vi "FRC_read utility images.vi"(7 "utilities data array":T1[](array[typedef])) -> (8 "menu array":cluster{"button":bool, "picture":picture}[](array[cluster]), 10 "names":string[](array[string]))   [LabVIEW 2023, in "GettingStartedWindow.lvlib"]
uses:
  <resource>/modes/FRC/GettingStartedWindow.lvlib
  <resource>/modes/FRC/FRC_UtilitiesData.ctl
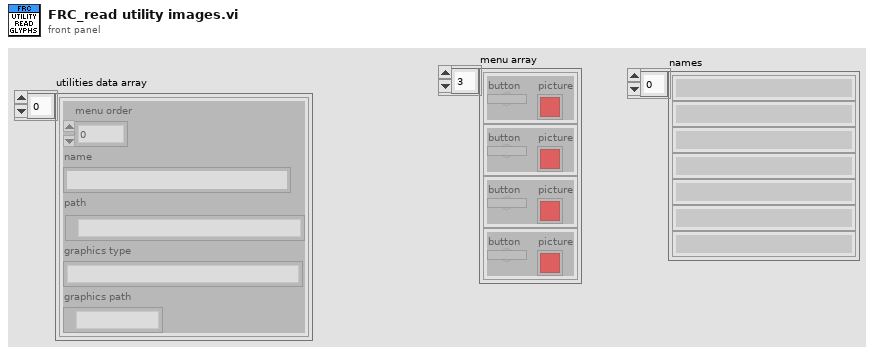
[diagram p1: front panel]
types:
  T1 = typedef "GettingStartedWindow.lvlib/FRC_UtilitiesData.ctl" = cluster{"menu order":i32, "name":string, "path":path, "graphics type":string, "graphics path":path}
  T2 = typedef "imagedata.ctl" = cluster{"image type":i32, "image depth":i32, "image":u8[], "mask":u8[], "colors":u32[], "Rectangle":cluster{"left":i16, "top":i16, "right":i16, "bottom":i16}}
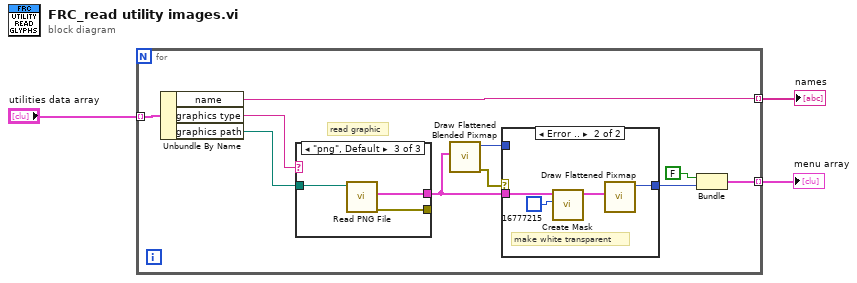
[diagram p0: block diagram]
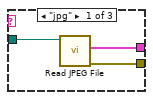
[diagram p3: hidden frame]
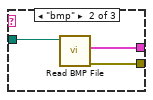
[diagram p4: hidden frame]
diagram:
  n1 = for {
    tunnel: "utilities data array" -> [w13] mode=indexing
    tunnel: [w9] -> w3 mode=indexing
    tunnel: [w8] -> w2 mode=indexing
    # "read graphic"
    n2 = Unbundle By Name(w13) -> ("name"=w9:string, "graphics type"=w12:string, "graphics path"=w11:path)
    n3 = case shown="\"png\", Default" w12 {
      tunnel: w11 -> [w21 w24 w27]
      tunnel: [w20 w23 w26] -> w7
      tunnel: [w19 w22 w25] -> _
      frame "jpg" {
        n4 = call <vilib>:"Read JPEG File.vi"("path to JPEG file"=w21) -> ("error out"=w19:errorcluster, "image data"=w20:T2)  [unwired: 8 in, 1 out]
      }
      frame "bmp" {
        n5 = call <vilib>:"Read BMP File.vi"("path to BMP file"=w24) -> ("error out"=w22:errorcluster, "image data"=w23:T2)  [unwired: 8 in, 1 out]
      }
      frame "png", Default {
        n6 = call <vilib>:"Read PNG File.vi"("path to PNG file"=w27) -> ("error out"=w25:errorcluster, "image data"=w26:T2)  [unwired: 8 in, 1 out]
      }
    }
    n7 = call <vilib>:"Draw Flattened Blended Pixmap.vi"("image data"=w7) -> ("error out"=w6:errorcluster, "new picture"=w4:picture)  [unwired: 7 in]
    n8 = case shown="Error .." w6 {
      tunnel: w7 -> [_ w16]
      tunnel: [w14 w15] -> w5
      tunnel: w4 -> [w14 _]
      frame No Error {
      }
      frame Error {
        # "make white transparent"
        n9 = call <vilib>:"Create Mask.vi"("Mask Color (Black)"=u32 16777215, "image data"=w16) -> ("image data"=w18:T2)  [unwired: 9 in]
        n10 = call <vilib>:"Draw Flattened Pixmap.vi"("image data"=w18) -> ("new picture"=w15:picture)  [unwired: 8 in]
      }
    }
    n11 = Bundle(FALSE, "new picture"=w5) -> (w8:cluster{bool, "new picture":picture})  [unwired: 1 in]
  }
  "menu array" <- w2
  "names" <- w3
